vi "Get Connection Status String.vi"(8 "error in (no error)":errorcluster, 11 "Modbus in":refnum<class "Modbus.lvclass">) -> (0 "error out":errorcluster, 2 "Status String":string, 3 "Modbus out":refnum<class "Modbus.lvclass">)   [LabVIEW 2026, in "Modbus.lvlib" / "Modbus.lvclass"]
uses:
  Modbus.lvclass
  Modbus.lvclass/Modbus.ctl
  Globals/Modbus Strings.vi
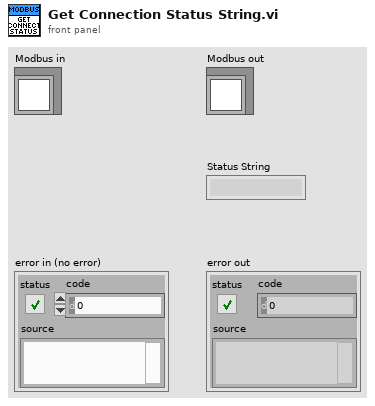
[diagram p1: front panel]
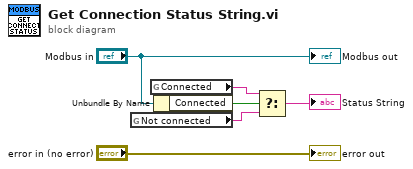
[diagram p0: block diagram]
diagram:
  n1 = global read "Modbus Strings.vi" "Not connected"() -> (w1:string)
  n2 = global read "Modbus Strings.vi" "Connected"() -> (w2:string)
  n3 = Unbundle By Name("Modbus in") -> ("Connected"=w3:bool)
  n4 = Select(t=w2, s=w3, f=w1) -> (s? t:f=→"Status String":string)
  "error out" <- "error in (no error)"
  "Modbus out" <- "Modbus in"
